vi "Register Events and Run.vi"(8 "error in (no error)":errorcluster, 11 "Panel in":refnum<class "Panel.lvclass">) -> (0 "error out":errorcluster, 2 "Panel Event Reg":refnum<event-registration>, 3 "Panel out":refnum<class "Panel.lvclass">)   [LabVIEW 2020, in "OOPanel.lvlib" / "Panel.lvclass"]
uses:
  Panel.lvclass
  Panel Events.ctl
  Visbility Event Data.ctl
  Visibility State.ctl
  Close Reason.ctl
  Panel.lvclass/Panel.ctl
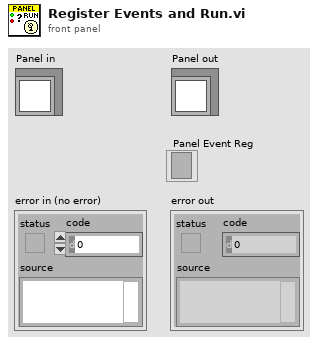
[diagram p1: front panel]
types:
  T1 = typedef "OOPanel.lvlib/Panel.lvclass/Panel Events.ctl" = cluster{"Visbility":refnum<user-event>, "Close":refnum<user-event>}
  T2 = typedef "OOPanel.lvlib/Panel.lvclass/Ref Data.ctl" = cluster{"Panel Ref":refnum<vi>, "SubPanel":refnum<vi>, "Close":bool, "Running":bool, "State":T3}
  T3 = typedef "OOPanel.lvlib/Panel.lvclass/Visibility State.ctl" = enum16{"Idle", "Closed", "Hidden", "Visible", "Subpanel"}
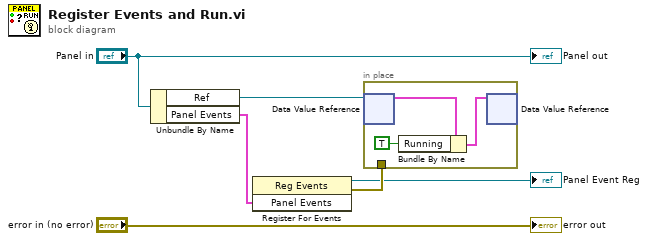
[diagram p0: block diagram]
diagram:
  n1 = Unbundle By Name("Panel in") -> ("Ref"=w5:refnum<data-value>, "Panel Events"=w3:T1)
  n2 = register-events(w3) -> (reference out=→"Panel Event Reg":refnum<event-registration>, error out=w2:errorcluster)  [unwired: 2 in]
  n3 = in-place {
    in-place-border: w2 -> [_]
    n4 = in-place-dvr #1(w5) -> (w9:T2)  [unwired: 1 out]
    n5 = Bundle By Name(cluster=w9, "Running"=TRUE) -> (w7:T2)
    n6 = in-place-dvr #1(w7) -> ()  [unwired: 2 out]
  }
  "error out" <- "error in (no error)"
  "Panel out" <- "Panel in"
